vi "Mark Document Dirty.vi"(8 "error in (no error)":errorcluster, 11 "Plugin Session in":refnum<class "Plugin Session.lvclass">) -> (0 "error out":errorcluster, 3 "Plugin Session out":refnum<class "Plugin Session.lvclass">)   [LabVIEW 2023, in "TLB` InstStu GPlugin Template.lvlib" / "InstrumentStudio Plugin SDK.lvlib" / "Plugin Session.lvclass"]
uses:
  Plugin Session.lvclass
  NationalInstruments.VIHost.Interop.dll
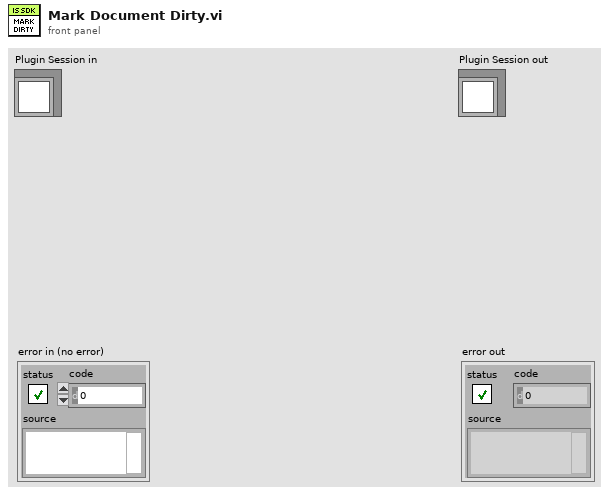
[diagram p1: front panel]
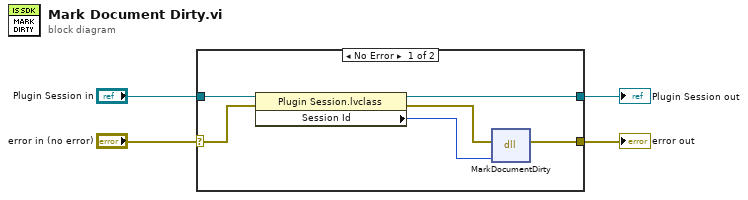
[diagram p0: block diagram]
diagram:
  n1 = case shown="No Error" "error in (no error)" {
    selector: "error in (no error)" -> [w8 w11]
    tunnel: "Plugin Session in" -> [w10 w12]
    tunnel: [w9 w12] -> w3
    tunnel: [w5 w11] -> w1
    frame No Error {
      n2 = property class="Plugin Session.lvclass"(reference=w10, error in=w8) -> (reference out=w9:refnum<class "Plugin Session.lvclass">, error out=w7:errorcluster, "Session Id"=w6:u64)
      n3 = dll-call lib="NationalInstruments.VIHost.Interop.dll" fn="MarkDocumentDirty"(error in=w7, "sessionId"=w6) -> (error out=w5:errorcluster)  [unwired: 4 in, 1 out]
    }
    frame Error {
    }
  }
  "Plugin Session out" <- w3
  "error out" <- w1
